vi "BuildVIPBFile.vi"(5 "vipb version":string, 7 "labview version":string, 8 "error in":errorcluster, 11 "path to vipb file":path) -> (0 "error out":errorcluster, 3 "build output":path)   [LabVIEW 2019]
uses:
  <vilib>/JKI/VIPM API/VIPM API_vipm_api.lvlib
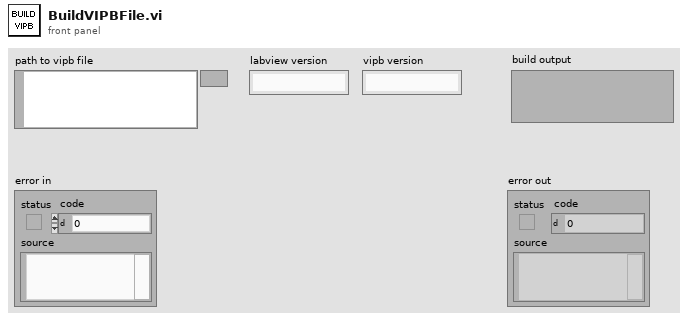
[diagram p1: front panel]
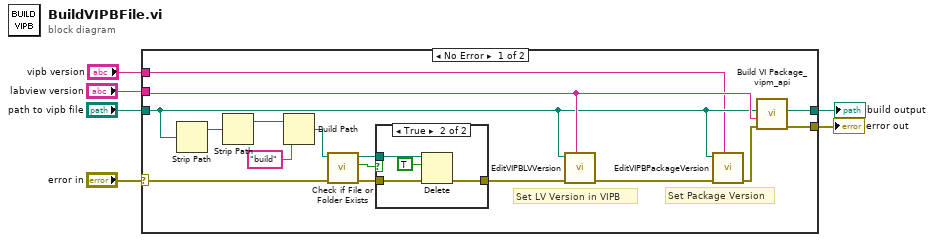
[diagram p0: block diagram]
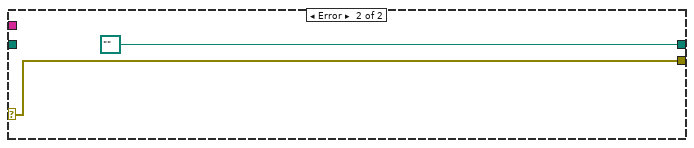
[diagram p3: hidden frame]
diagram:
  n1 = case shown="No Error" "error in" {
    selector: "error in" -> [w15 w28]
    tunnel: "path to vipb file" -> [w9 _]
    tunnel: [w21 path "" ("Build Output")] -> w6
    tunnel: [w20 w28] -> w5
    tunnel: "labview version" -> [w11 _]
    tunnel: "vipb version" -> [w8 _]
    frame No Error {
      # "Set Package Version"
      # "Set LV Version in VIPB"
      n2 = Strip Path(path=w9) -> (stripped path=w19:path)  [unwired: 1 out]
      n3 = Strip Path(path=w19) -> (stripped path=w13:path)  [unwired: 1 out]
      n4 = Build Path(base path=w13, name or relative path="build") -> (appended path=w16:path)
      n5 = call <vilib>:"Check if File or Folder Exists.vi"("error in (no error)"=w15, "path"=w16) -> ("error out"=w14:errorcluster, "file or folder exists?"=w17:bool)  [unwired: 7 in, 1 out]
      n6 = case shown="True" w17 {
        tunnel: w16 -> [_ w26]
        tunnel: w14 -> [w22 w25]
        tunnel: [w22 w24] -> w12
        frame False {
        }
        frame True {
          n7 = Delete(path (use dialog)=w26, entire hierarchy (F)=TRUE, error in=w25) -> (error out=w24:errorcluster)  [unwired: 2 in, 2 out]
        }
      }
      n8 = call "EditVIPBLVVersion.vi"("labview version"=w11, "error in"=w12, "path to vipb file"=w9) -> ("error out"=w10:errorcluster)  [unwired: 8 in]
      n9 = call "EditVIPBPackageVersion.vi"("package version"=w8, "error in"=w10, "path to vipb file"=w9) -> ("error out"=w7:errorcluster)  [unwired: 8 in]
      n10 = call <vilib>:"Build VI Package_vipm_api.vi"("error in (no error)"=w7, "LabVIEW Version"=w11, "Path to VIPB File"=w9) -> ("error out"=w20:errorcluster, "Build Output"=w21:path)  [unwired: 7 in]
    }
    frame Error {
    }
  }
  "build output" <- w6
  "error out" <- w5
